vi "Read TAI Start Time (ns).vi"(8 "error in (no error)":errorcluster, 11 "XNET CAN RW in":refnum<class "XNET CAN RW.lvclass">) -> (0 "error out":errorcluster, 2 "TAI Start Time (ns)":i64, 3 "XNET CAN RW out":refnum<class "XNET CAN RW.lvclass">)   [LabVIEW 2021, in "XNET CAN RW.lvclass"]
uses:
  XNET CAN RW.lvclass
  XNET CAN RW.lvclass/XNET CAN RW.ctl
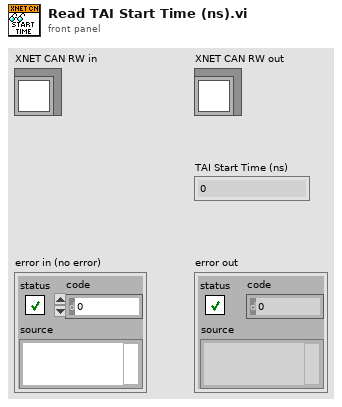
[diagram p1: front panel]
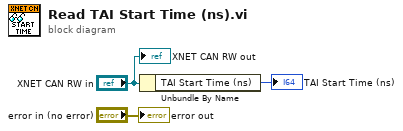
[diagram p0: block diagram]
diagram:
  n1 = Unbundle By Name("XNET CAN RW in") -> ("TAI Start Time (ns)"=→"TAI Start Time (ns)":i64)
  "error out" <- "error in (no error)"
  "XNET CAN RW out" <- "XNET CAN RW in"
